vi "WindTurbineMenu.vi"(0 "ip":string) -> ()   [LabVIEW 2024]
panel:
  in  "Speed":dbl(slide) step=1.0 scale=64.0..255.0 scale format="%#.6g"
  in  "Cancel Button":bool
  in  "OK Button":bool
  # "WindTurbine Setting Menu"
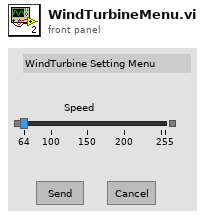
[diagram p1: front panel]
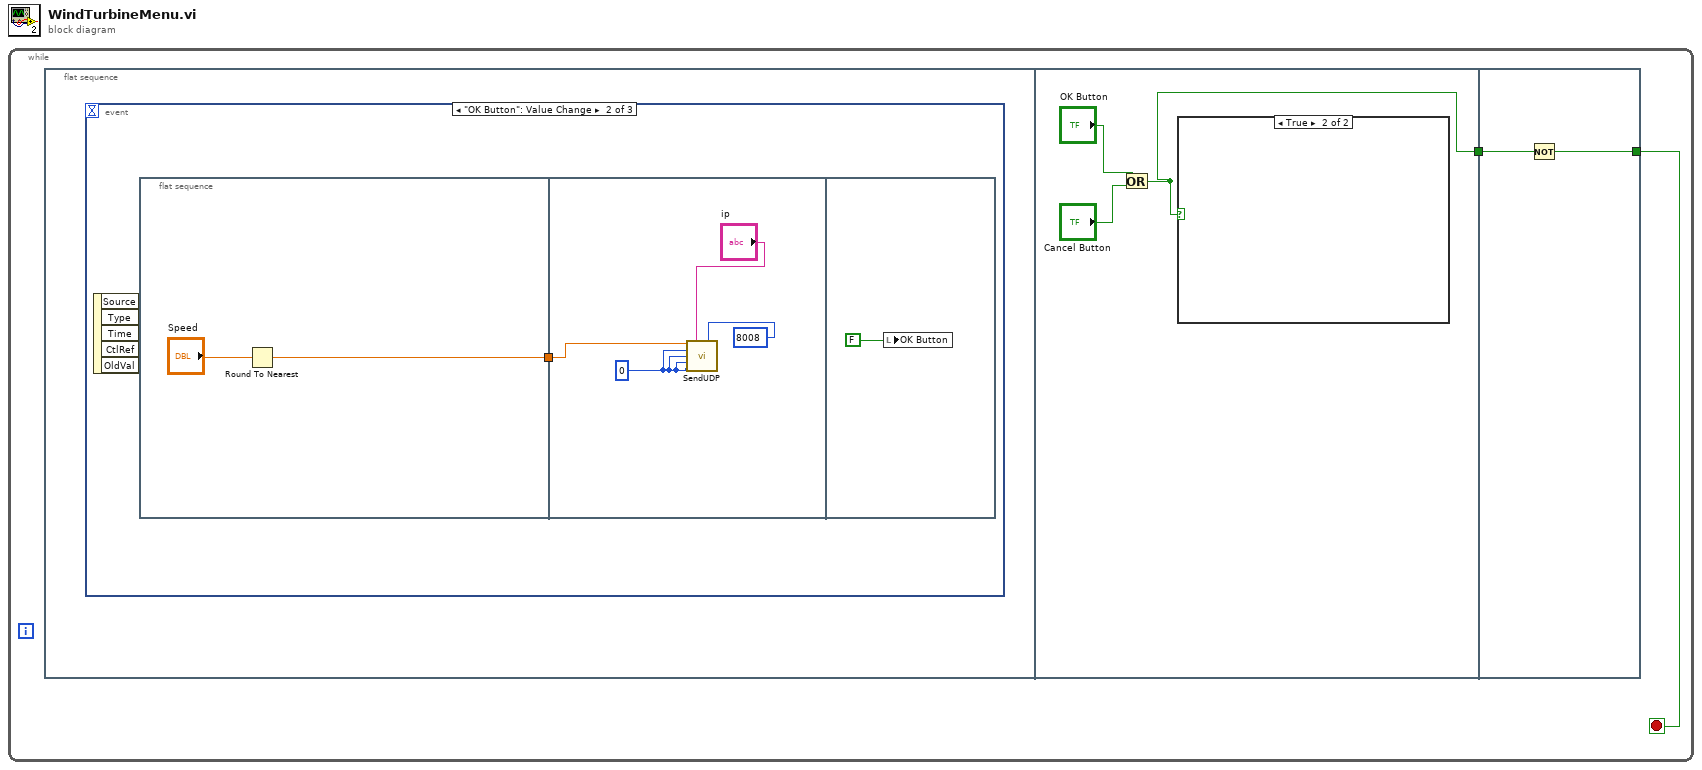
[diagram p0: block diagram]
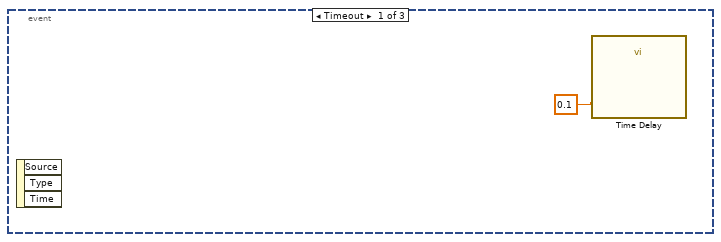
[diagram p2: hidden frame]
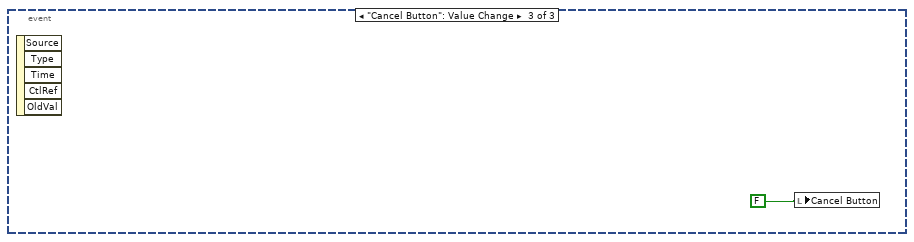
[diagram p3: hidden frame]
diagram:
  n1 = while {
    stop <- w2 stop-if-true
    n2 = flat-sequence {
      tunnel: [w13] -> w1
      tunnel: [w17] -> w2
      tunnel: w1 -> [w16]
      frame #0 {
        n3 = event shown="[1] \"OK Button\": Value Change" {
          selector: _ -> [_ _ _]
          dyn-events: _ -> [_ _ _]
          timeout: _ -> [_ _ _]
          event Timeout {
            n4 = event-data() -> ()  [unwired: 1 in, 3 out]
            n5 = call "Time Delay"("Delay Time (s)"=0.1) -> ()  [unwired: 10 in, 1 out]
          }
          event "OK Button": Value Change {
            n6 = event-data() -> ()  [unwired: 1 in, 5 out]
            n7 = flat-sequence {
              tunnel: [w5] -> w4
              tunnel: w4 -> [w8]
              frame #0 {
                n8 = Round To Nearest(number="Speed") -> (nearest integer value=w5:dbl)
              }
              frame #1 {
                w7 = u8 0 ("Arg7")
                n9 = call "SendUDP.vi"("Arg3"=w8, "IP"="ip", "Port"=8008, "Arg4"=w7, "Arg5"=w7, "Arg6"=w7, "Arg7"=w7) -> ()  [unwired: 9 in]
              }
              frame #2 {
                n10 = local write "OK Button"(FALSE ("OK Button")) -> ()
              }
            }
          }
          event "Cancel Button": Value Change {
            n11 = event-data() -> ()  [unwired: 1 in, 5 out]
            n12 = local write "Cancel Button"(FALSE ("Cancel Button")) -> ()
          }
        }
      }
      frame #1 {
        n13 = Or(x="OK Button", y="Cancel Button") -> (x .or. y?=w13:bool)
        n14 = case shown="True" w13 {
          frame False {
          }
          frame True {
          }
        }
      }
      frame #2 {
        n15 = Not(x=w16) -> (.not. x?=w17:bool)
      }
    }
  }
